vi "Query Motor Status.vi"(8 "error in (no error)":errorcluster, 11 "CO3000 in":refnum<class "CO3000.lvclass">) -> (0 "error out":errorcluster, 2 "Motor Stop?":bool, 3 "CO3000 out":refnum<class "CO3000.lvclass">)   [LabVIEW 2023, in "Turn Table and Mast.lvlib" / "CO3000.lvclass"]
uses:
  CO3000.lvclass
  CO3000.lvclass/CO3000.ctl
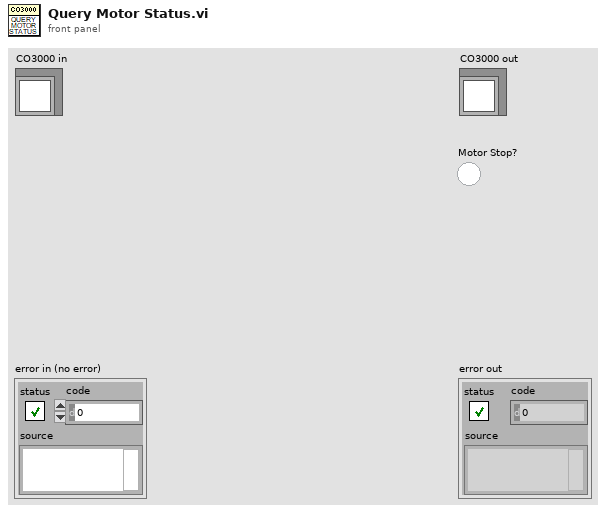
[diagram p1: front panel]
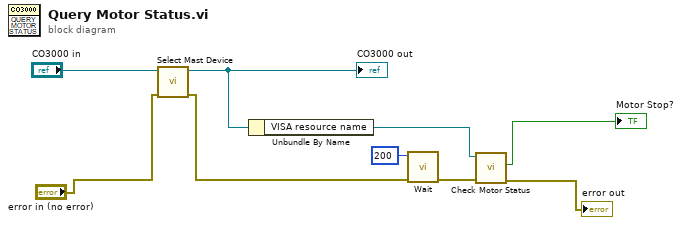
[diagram p0: block diagram]
diagram:
  n1 = call "Select Mast Device.vi"("error in (no error)"="error in (no error)", "CO3000 in"="CO3000 in") -> ("error out"=w1:errorcluster, "CO3000 out"=w3:refnum<class "CO3000.lvclass">)  [unwired: 8 in]
  "CO3000 out" <- w3
  n2 = Unbundle By Name(w3) -> ("VISA resource name"=w8:refnum<visa-resource-name>)
  n3 = call "Wait.vi"("에러 상수 입력"=w1, "대기 시간 (ms)"=u32 200) -> ("에러 상수 출력"=w7:errorcluster)  [unwired: 9 in]
  n4 = call "Check Motor Status.vi"("error in (no error)"=w7, "VISA Refnum in"=w8) -> ("error out"=→"error out":errorcluster, "Motor Stop?"=→"Motor Stop?":bool)  [unwired: 7 in, 1 out]
